vi "Run.vi"(8 "error in (no error)":errorcluster, 10 "UI Refs":T1, 11 "H1Velocity":refnum<class "H1 Velocity.lvclass">) -> (0 "error out":errorcluster, 3 "H1Velocity out":refnum<class "H1 Velocity.lvclass">)   [LabVIEW 2025, in "H1 Plotter.lvlib" / "H1 Velocity.lvclass"]
uses:
  H1 Velocity.lvclass
  Users/Public/Documents/Sandia National Labs/TSS Plugin/Tests/XY Plotter.lvlibp/XY Plotter configuration/XY Plotter configuration.lvclass
  H1 Velocity.lvclass/H1 Velocity.ctl
  Users/Public/Documents/Sandia National Labs/TSS Plugin/Tests/XY Plotter.lvlibp/XY Plotter configuration/Read XY Plotter.vi
  Users/Public/Documents/Sandia National Labs/TSS Plugin/CEF.lvlibp/serializable configuration/CEF_serializable configuration.lvclass
  Users/Public/Documents/Sandia National Labs/TSS Plugin/Tests/XY Plotter.lvlibp/XY  Plotter/XY Plotter.lvclass
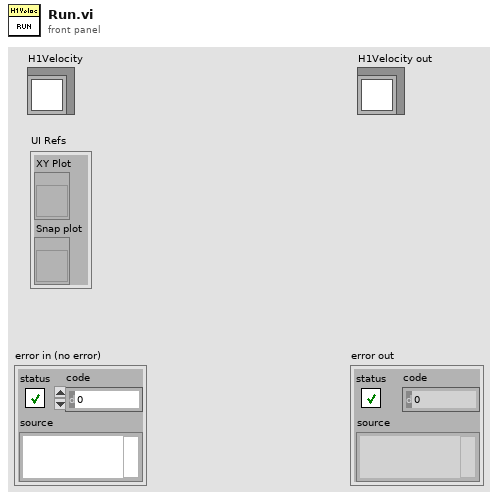
[diagram p1: front panel]
types:
  T1 = cluster{"XY Plot":refnum<vi>, "Snap plot":refnum<vi>}
  T2 = typedef "XY Plotter.lvlibp/XY Plotter configuration.lvclass/XY Plotter.ctl" = cluster{"Data Rate":i32, "Y-Scales":cluster{"Label":string, "Max":dbl, "Min":dbl, "Unit":enum16{"---", "V", "mA", "sec", "dB", "deg", "in/s", "in", "lbf", "Hz", "psi", "gpm"}, "Visible":bool}[], "Note":string, "History Length":i32, "DataLog Path":path, "Plot type":bool, "X-Scales":cluster{"Label":string, "Max":dbl, "Min":dbl, "Unit":enum16{"---", "V", "mA", "sec", "dB", "deg", "in/s", "in", "lbf", "Hz", "psi", "gpm"}, "Visible":bool}[], "Plot List":cluster{"Plot Name":string, "X Scale Index":u32, "Y Scale Index":u32, "Visible":bool}[]}
  T3 = cluster{"Plot Name":string, "X Scale Index":u32, "Y Scale Index":u32, "Visible":bool}[]
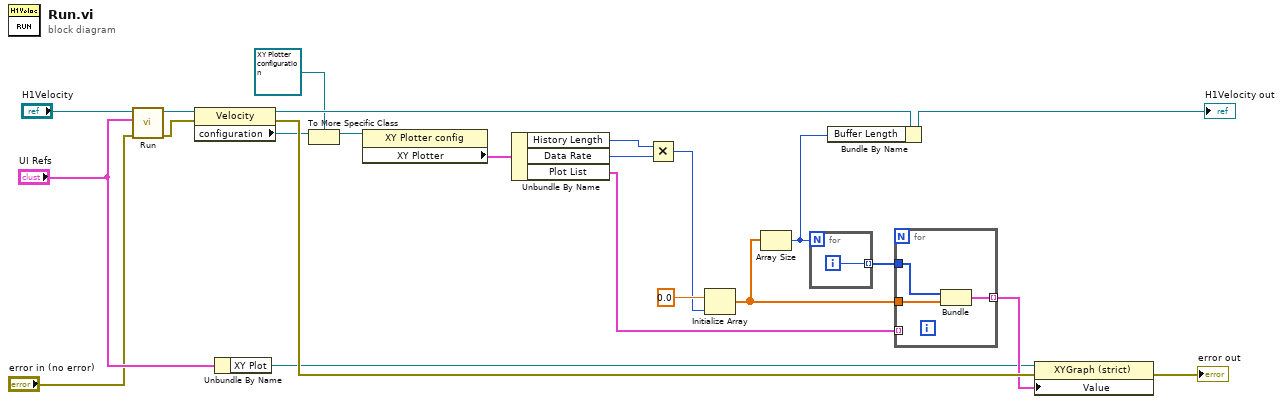
[diagram p0: block diagram]
diagram:
  n1 = call-parent "Run.vi"("error in (no error)"="error in (no error)", "UI Refs"="UI Refs", "XY Plotter"="H1Velocity") -> ("error out"=w1:errorcluster, "XY Plotter out"=w4:refnum<class "H1 Velocity.lvclass">)  [unwired: 7 in]
  n2 = property class="Velocity"(reference=w4, error in=w1) -> (reference out=w21:refnum<class "H1 Velocity.lvclass">, error out=w22:errorcluster, "configuration"=w7:refnum<class "CEF_serializable configuration.lvclass">)
  n3 = Unbundle By Name("UI Refs") -> ("XY Plot"=w8:refnum<vi>)
  n4 = To More Specific Class(target class=refnum<class "XY Plotter configuration.lvclass"> refnum ("XY Plotter.lvlibp:XY Plotter config"), reference=w7) -> (specific class reference=w5:refnum<class "XY Plotter configuration.lvclass">)  [unwired: 1 in, 1 out]
  n5 = property class="XY Plotter config"(reference=w5) -> ("XY Plotter"=w20:T2)  [unwired: 1 in, 2 out]
  n6 = Unbundle By Name(w20) -> ("History Length"=w17:i32, "Data Rate"=w18:i32, "Plot List"=w9:T3)
  n7 = Multiply(x=w17, y=w18) -> (x*y=w16:i32)
  n8 = Initialize Array(0.0 ("element"), w16) -> (w15:dbl[])
  n9 = Array Size(array=w15) -> (size(s)=w12:i32)
  n10 = for {
    N: w12 -> [_]
    tunnel: [w24] -> w14 mode=indexing
    i -> [w24]
  }
  n11 = Bundle By Name(cluster=w21, "Buffer Length"=w12) -> (→"H1Velocity out":refnum<class "H1 Velocity.lvclass">)
  n12 = for {
    tunnel: w9 -> [_] mode=indexing
    tunnel: w15 -> [w27]
    tunnel: [w26] -> w13 mode=indexing
    tunnel: w14 -> [w25]
    n13 = Bundle(w25, w27) -> (w26:cluster{i32[], dbl[]})  [unwired: 1 in]
  }
  n14 = property class="XYGraph (strict)"(reference=w8, error in=w22, "Value"=w13) -> (error out=→"error out":errorcluster)  [unwired: 1 out]
